vi "get_value_for_integer.vi"(8 "error in (no error)":errorcluster, 11 "Value in":refnum<class "Value.lvclass">) -> (0 "error out":errorcluster, 3 "integer_value":i64)   [LabVIEW 2020, in "toml_edit.lvlib" / "Value.lvclass"]
uses:
  Value.lvclass
  value_type--enum.ctl
  Value.lvclass/Value.ctl
  dragon_toml_64.dll
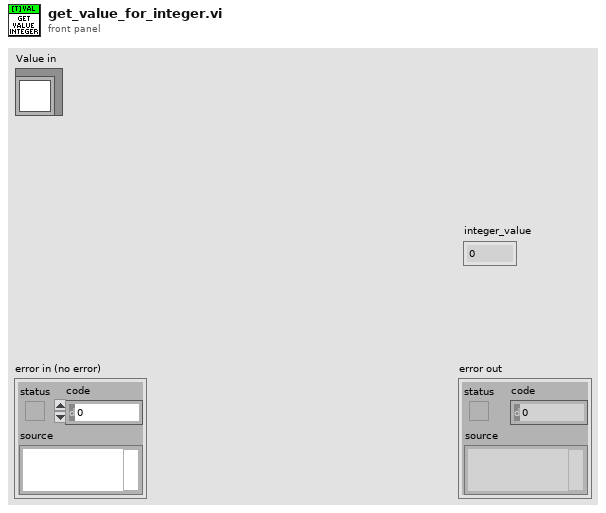
[diagram p1: front panel]
types:
  T1 = typedef "toml_edit.lvlib/Value.lvclass/value_type--enum.ctl" = enum16{"Unknown", "String", "Integer", "Float", "Boolean", "Datetime", "Array", "InlineTable"}
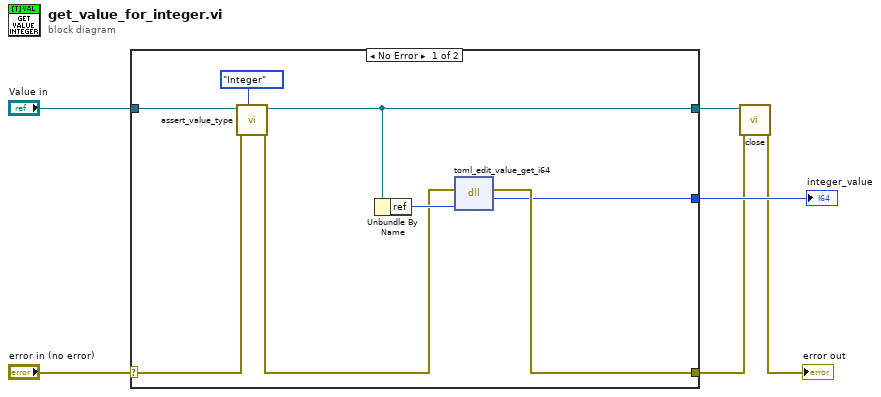
[diagram p0: block diagram]
diagram:
  n1 = case shown="No Error" "error in (no error)" {
    selector: "error in (no error)" -> [w8 w16]
    tunnel: [w14 w16] -> w2
    tunnel: [w9 w15] -> w3
    tunnel: "Value in" -> [w10 w15]
    tunnel: [w12 _] -> w4
    frame No Error {
      n2 = call "assert_value_type.vi"("value_type"=value_type--enum."Integer", "error in (no error)"=w8, "Value in"=w10) -> ("error out"=w7:errorcluster, "Value out"=w9:refnum<class "Value.lvclass">)  [unwired: 7 in]
      n3 = Unbundle By Name(w9) -> ("ref"=w13:u64)
      n4 = dll-call lib="C:/projects/dragon-desktop/source/submodules/toml-edit-labview/lv_src/dragon_toml_*.*" fn="toml_edit_value_get_i64"(error in=w7, "item_ref"=w13) -> (error out=w14:errorcluster, "i64_value"=w12:i64)  [unwired: 3 in, 1 out]
    }
    frame Error {
    }
  }
  "integer_value" <- w4
  n5 = call "close.vi"("error in (no error)"=w2, "Value in"=w3) -> ("error out"=→"error out":errorcluster)  [unwired: 9 in]
